vi "VIH Utility - FILE - Create Directory.vi"(6 "error in":errorcluster, 9 "directory path":path=path "") -> (0 "error out":errorcluster, 1 "new created":bool, 3 "directory path out":path)   [LabVIEW 2014]
doc: "::: VI Helpeks :::\nCopyright (c) 2000-2026 Konstantin Shifershteyn. All rights reserved."
panel:
  # "VI Helpeks\nCopyright (c) 2012-2026 Konstantin Shifershteyn"
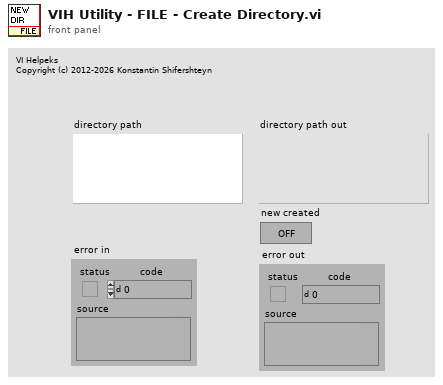
[diagram p1: front panel]
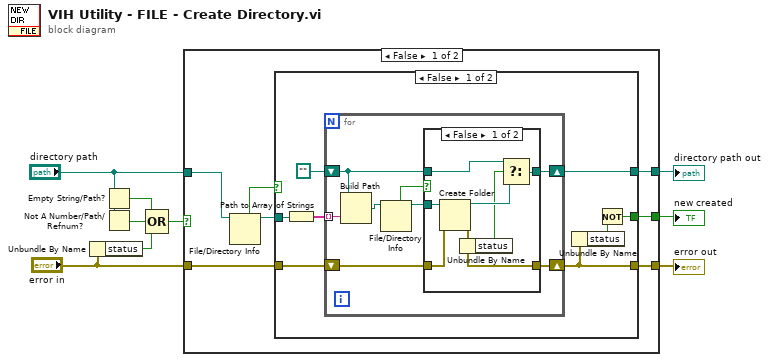
[diagram p0: block diagram]
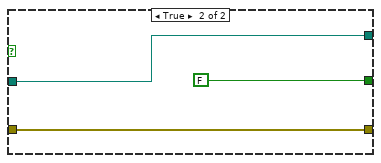
[diagram p3: hidden frame]
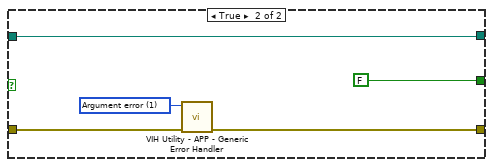
[diagram p4: hidden frame]
diagram:
  n1 = Unbundle By Name("error in") -> ("status"=w1:bool)
  n2 = Empty String/Path?(string/path="directory path") -> (empty?=w3:bool)
  n3 = Not A Number/Path/Refnum?(number/path/refnum="directory path") -> (NaN/Path/Refnum?=w4:bool)
  n4 = Compound Arithmetic op=OR(w3, w4, w1) -> (w2:bool)
  n5 = case shown="False" w2 {
    tunnel: [w14 w48] -> w9
    tunnel: "error in" -> [w12 w47]
    tunnel: [w13 w46] -> w8
    tunnel: [w11 FALSE] -> w6
    tunnel: "directory path" -> [w10 w48]
    frame False {
      n6 = File/Directory Info(path=w10) -> (path out=w15:path, directory=w16:bool)  [unwired: 1 in, 5 out]
      n7 = case shown="False" w16 {
        tunnel: w15 -> [w24 w42]
        tunnel: [w21 w42] -> w14
        tunnel: w12 -> [w20 w44]
        tunnel: [w19 w44] -> w13
        tunnel: [w17 FALSE] -> w11
        frame False {
          n8 = Path to Array of Strings(0:w24) -> (2:w23:string[])  [unwired: 1 out]
          n9 = for {
            tunnel: w23 -> [w32] mode=indexing
            shift-right: [w30] -> w21
            shift-left: path "" -> [w27]
            shift-right: [w25] -> w19
            shift-left: w20 -> [w26]
            n10 = Build Path(base path=w27, name or relative path=w32) -> (appended path=w29:path)
            n11 = File/Directory Info(path=w29) -> (path out=w28:path, directory=w31:bool)  [unwired: 1 in, 5 out]
            n12 = case shown="False" w31 {
              tunnel: [w36 w41] -> w30
              tunnel: w28 -> [w39 w41]
              tunnel: w27 -> [w34 _]
              tunnel: w26 -> [w38 w40]
              tunnel: [w37 w40] -> w25
              frame False {
                n13 = Create Folder(path (use dialog)=w39, error in=w38) -> (created path=w35:path, error out=w37:errorcluster)  [unwired: 2 out]
                n14 = Unbundle By Name(w37) -> ("status"=w33:bool)
                n15 = Select(t=w34, s=w33, f=w35) -> (s? t:f=w36:path)
              }
              frame True {
              }
            }
          }
          n16 = Unbundle By Name(w19) -> ("status"=w18:bool)
          n17 = Not(x=w18) -> (.not. x?=w17:bool)
        }
        frame True {
        }
      }
    }
    frame True {
      w45 = 1 items=["No error", "Argument error", "Memory is full", "Out of zone", "End of file", "File already open", "Generic file I/O error", "File not found", "File permission error", "Disk is full", "Duplicate path", "Too many files open", "System feature not enabled", "Resource file not found", "Cannot add resource", "Resource not found", "Image not found", "Image memory error", "Pen does not exist", "Config type invalid", "Config token not found", "Config parse error", "Config memory error", "Bad external code format", "Bad external code offset", "External code not present", "Null window", "Destroy window error", "Null menu", "Print aborted", "Bad print record", "Print driver error", "Windows error during printing", "Memory error during printing", "Print dialog error", "Generic print error", "Invalid device refnum", "Device not found", "Device parameter error", "Device unit error", "Cannot open device", "Device call aborted", "Generic error", "Cancelled by user", "Object ID too low", "Object ID too high", "Object not in heap", "Unknown heap", "Unknown object (invalid DefProc)", "Unknown object (DefProc not in table)", "Message out of range", "Invalid (null) method", "Unknown message", "Manager call not supported", "Bad address", "Network operation in progress", "Network operation timed out", "Connection is busy", "Network attribute not supported", "Network error", "Address in use", "System out of memory", "Connection aborted", "Connection refused", "Not connected", "Already connected", "Connection closed", "Initialization error (interapplication manager)", "Bad occurrence", "Wait on unbound occurrence handler", "Occurrence queue overflow", "Datalog type conflict", "Unused", "Unrecognized type (interapplication manager)", "Memory corrupt", "Failed to make temporary DLL", "Old CIN version", "Drag socket not found", "Failed to load drop-object", "Failed to register OLE object", "Failed to release OLE object", "Format specifier type mismatch", "Unknown format specifier", "Too few format specifiers", "Too many format specifiers", "Scan failed", "Newer CIN version", "Error converting to variant", "Runtime menu error", "Password tampered", "Variant attribute not found", "Incompatible variant data type", "Event data is not available", "Event Store is not present", "Occurrence is not found", "Event Queue is not created", "Event info is not available", "Refnum passed is NULL", "Error retrieving Class GUID", "Error retrieving CoClass GUID", "Error retrieving TypeLib GUID.", "Bad built application magic bytes.", "Specific driver is different from the specific driver associated with the Logical Name.", "There is no session opened to the class driver.", "Max Error", "MAX - Error with config objects", "MAX - Error loading configuration", "MAX - Group not supported"]
      n18 = call "VIH Utility - APP - Generic Error Handler.vi"("error in"=w47, "error code"=w45) -> ("error out"=w46:errorcluster)  [unwired: 9 out]
    }
  }
  "directory path out" <- w9
  "error out" <- w8
  "new created" <- w6
